vi "Restore Request ID.vi"(8 "error in":errorcluster, 10 "response":string, 11 "request":string) -> (0 "error out":errorcluster, 3 "response out":string)   [LabVIEW 2020, in "MCP Server.lvlib"]
doc: "Makes a JSON-RPC response carry the id of its request exactly as the client sent it, and makes sure a notification is never answered.\n\nThe request handlers read the id as a 32 bit integer, so a string id or a large or fractional number would come back changed. This VI copies the raw id item of the request into the response.\n\n- request has a top-level id: a non-empty response gets that id as raw JSON (a string stays a string, a number stays the same number). An empty response stays empty.\n- request has no id but has a method (a notification): response out is empty, whatever the handler produced.\n- request has neither (not a valid message): the response is passed through unchanged, so a parse error keeps id null."
uses:
  MCP Server.lvlib
  <vilib>/JDP Science/JSONtext/Next JSON Value.vi
  <vilib>/JDP Science/JSONtext/String Subset.vi
  <vilib>/JDP Science/JSONtext/Parsing/Advance past next JSON Value (inlined COPY).vi
  <vilib>/JDP Science/JSONtext/Parsing/Advance past whitespace.vi
  <vilib>/JDP Science/JSONtext/Parsing/Advance past String.vi
  <vilib>/JDP Science/JSONtext/Parsing/Advance past Number.vi
  <vilib>/JDP Science/JSONtext/Parsing/Advance past Line Ending.vi
  <vilib>/JDP Science/JSONtext/Parsing/Parse Full Path or Item Name.vi
  <vilib>/JDP Science/JSONtext/Parsing/Advance past Array.vi
  <vilib>/JDP Science/JSONtext/Parsing/Advance past Object.vi
  <vilib>/JDP Science/JSONtext/support/Error Cluster From Code.vi
  <vilib>/JDP Science/JSONtext/Offset/Find Item Locations by Path.vi
  <vilib>/JDP Science/JSONtext/JSONtext.lvlib
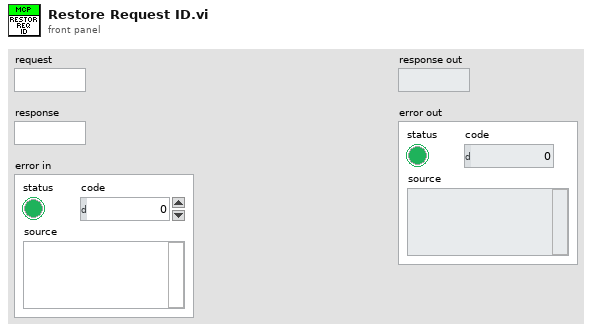
[diagram p1: front panel]
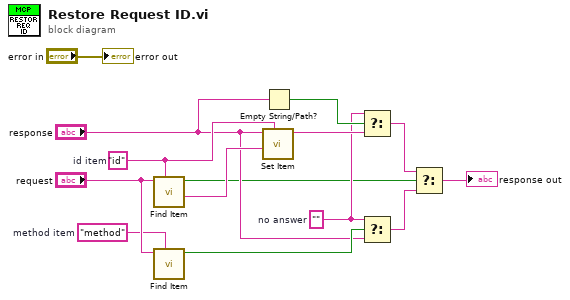
[diagram p0: block diagram]
diagram:
  w8 = ""  # no answer
  w13 = "method"  # method item
  w12 = "id"  # id item
  n1 = call <vilib>:"Find Item.vi"("$Path or Item Name"=w12, "JSON"="request") -> ("<JSON>"=w11:string, "Found"=w4:bool)  [unwired: 6 in, 2 out]
  n2 = call <vilib>:"Find Item.vi"("$Path or Item Name"=w13, "JSON"="request") -> ("Found"=w7:bool)  [unwired: 6 in, 3 out]
  n3 = call <vilib>:"Set Item.vi"("$Path or Item Name"=w12, "JSON to Insert"=w11, "JSON"="response") -> ("<JSON>"=w9:string)  [unwired: 5 in, 2 out]
  n4 = Empty String/Path?(string/path="response") -> (empty?=w10:bool)
  n5 = Select(t=w8, s=w10, f=w9) -> (s? t:f=w5:string)
  n6 = Select(t=w8, s=w7, f="response") -> (s? t:f=w3:string)
  n7 = Select(t=w5, s=w4, f=w3) -> (s? t:f=→"response out":string)
  "error out" <- "error in"
